vi "FuncVI-lvErrorMessage.vi"(5 "InstanceRef":T2, 9 "arg list":T1[](array[typedef]) {"num" format="%.2f"}) -> (0 "error out":bool, 3 "result":T1 {"num" format="%.2f"})   [LabVIEW 2021]
doc: "::: CalcExpress Toolkit :::\nCopyright (c) 2000-2026 Konstantin Shifershteyn. All rights reserved."
uses:
  cetypes.llb/CalcExpress Function Argument Info.ctl
  cetypes.llb/CalcExpress Instance RefNum.ctl
panel:
  in  "max arg num":i32=2
  in  "min arg num":i32
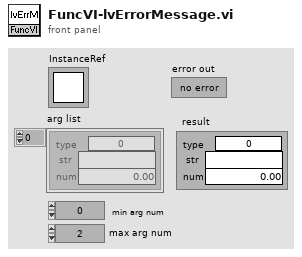
[diagram p1: front panel]
types:
  T1 = typedef "CalcExpress Function Argument Info.ctl" = cluster{"type":u32, "str":string, "num":dbl}
  T2 = typedef "CalcExpress Instance RefNum.ctl" = refnum<k1>
  T3 = cluster{"index":i32, "data type":enum32{"String", "DBL Number", "identifier", "1D Array of DBL", "2D Array of DBL", "CDB Number", "1D Array of CDB", "2D Array of CDB", "1D Array of String", "2D Array of String", "Unknown data type"}, "default num":dbl, "default str":string}
  T4 = enum32{"String", "DBL Number", "identifier", "1D Array of DBL", "2D Array of DBL", "CDB Number", "1D Array of CDB", "2D Array of CDB", "1D Array of String", "2D Array of String", "Unknown data type"}
  T5 = cluster{"index":i32, "data type":enum32{"String", "DBL Number", "identifier", "1D Array of DBL", "2D Array of DBL", "CDB Number", "1D Array of CDB", "2D Array of CDB", "1D Array of String", "2D Array of String", "Unknown data type"}, "default num":dbl, "default str":string}[]
  T6 = cluster{"data type":enum32{"String", "DBL Number", "identifier", "1D Array of DBL", "2D Array of DBL", "CDB Number", "1D Array of CDB", "2D Array of CDB", "1D Array of String", "2D Array of String", "Unknown data type"}, string, dbl}
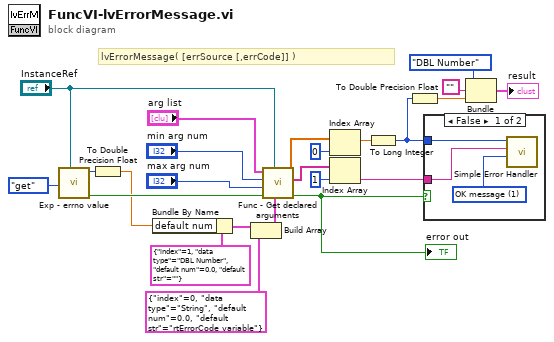
[diagram p0: block diagram]
diagram:
  # "lvErrorMessage( [errSource [,errCode]] )"
  n1 = call "Exp - errno value.vi"("InstanceRef"="InstanceRef", "action"=enum32{"get", "set"}."get") -> ("error out"=w5:bool, "errno value out"=w15:i32)  [unwired: 5 in, 1 out]
  n2 = To Double Precision Float(number=w15) -> (double precision float=w3:dbl)
  n3 = Bundle By Name(cluster=T3 {"index"=1, "data type"=enum."DBL Number", "default num"=0.0, "default str"=""} ("arg descriptor"), "default num"=w3) -> (w8:T3)
  n4 = Build Array(w8, T3 {"index"=0, "data type"=enum."String", "default num"=0.0, "default str"="rtErrorCode variable"} ("arg descriptor")) -> (w6:T5)
  n5 = call "Func - Get declared arguments.vi"("arg descriptors"=w6, "InstanceRef"="InstanceRef", "error in"=w5, "max arg num"="max arg num", "min arg num"="min arg num", "arg list"="arg list") -> ("error out"=w23:bool, "str list"=w12:string[], "num list"=w14:dbl[])  [unwired: 2 in, 1 out]
  "error out" <- w23
  n6 = Index Array(array=w14, index=0) -> (element=w10:dbl)
  n7 = Index Array(array=w12, index=1) -> (element=w18:string)
  n8 = To Long Integer(number=w10) -> (32bit integer=w20:i32)
  n9 = To Double Precision Float(number=w20) -> (double precision float=w17:dbl)
  n10 = case shown="False" w23 {
    tunnel: w20 -> [w25 _]
    tunnel: w18 -> [w26 _]
    frame False {
      w27 = 1 items=["no dialog", "OK message", "continue or stop message"] ("type of dialog (OK msg:1)")
      n11 = call <vilib>:"Simple Error Handler.vi"("error code (no error:0)"=w25, "error source (\" \")"=w26, "type of dialog (OK msg:1)"=w27) -> ()  [unwired: 2 in, 5 out]
    }
    frame True {
    }
  }
  n12 = Bundle("data type"=T4."DBL Number", "", w17) -> (→"result":T6)  [unwired: 1 in]
